vi "Unicode Languages to HEX-String Array.vi"(11 "Config Data in":T1) -> (3 "Config Data out":T1)   [LabVIEW 2019, in "Language Selection.lvlib"]
doc: "- - -\nCopyright (c) 2026, Merecs Engineering GmbH"
uses:
  Language Selection.lvlib
  TypeDefs/Cluster Language Configuration.ctl
  Cluster Settings Data.ctl
  TypeDefs/Cluster Language.ctl
  TypeDefs/Cluster PropertyTranslation.ctl
  TypeDefs/Enum Property Type.ctl
panel:
  # "Connector Pane"
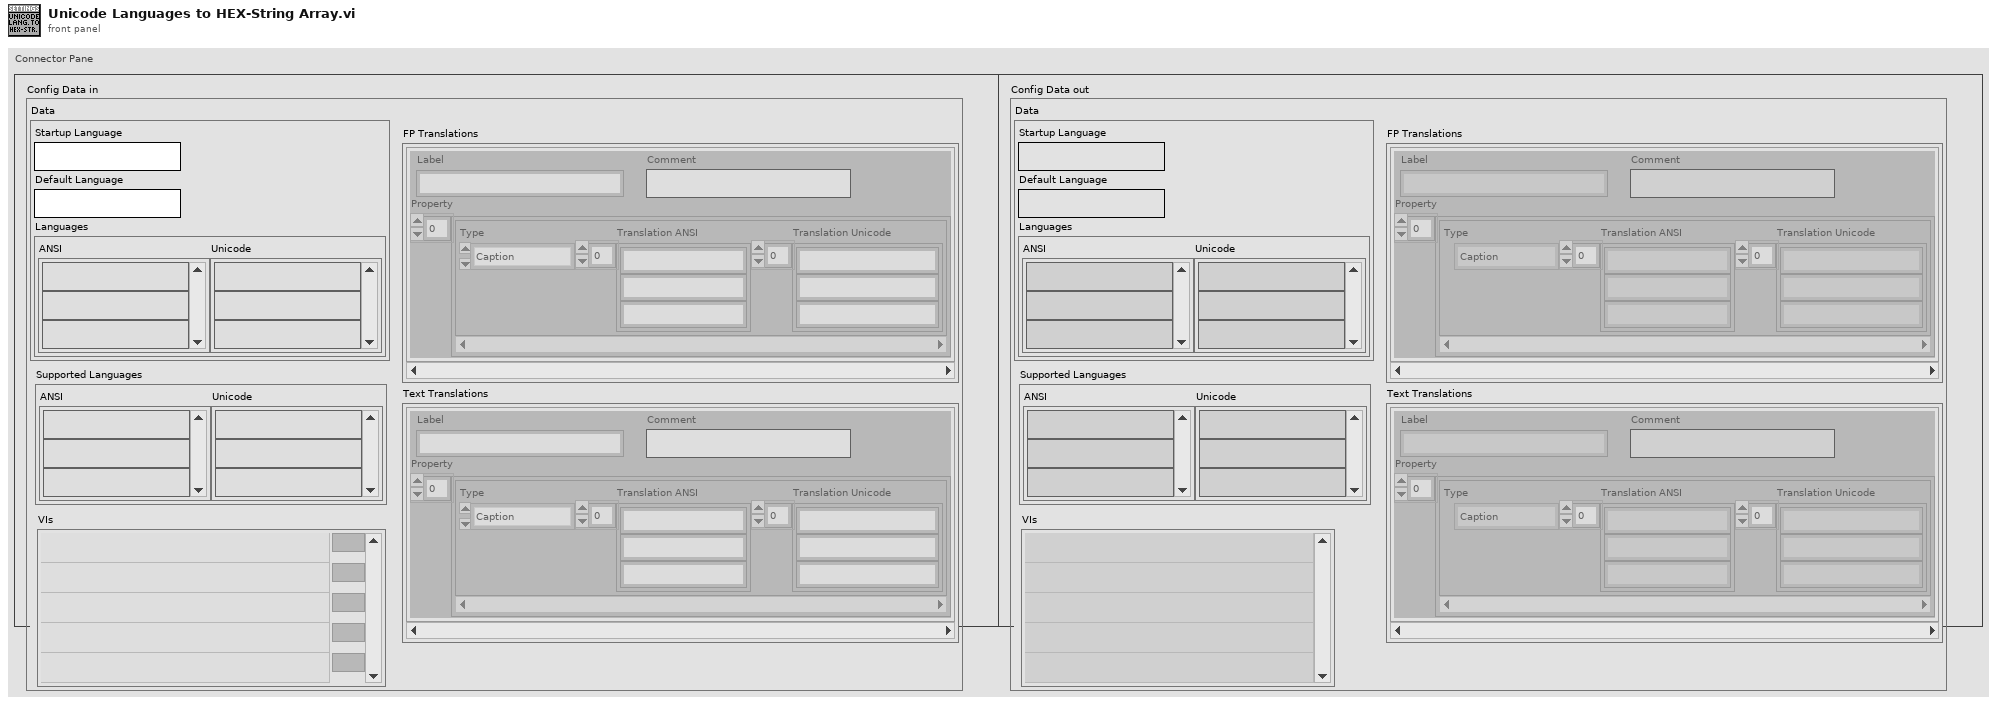
[diagram p1: front panel]
types:
  T1 = typedef "Language Selection.lvlib/Cluster Language Configuration.ctl" = cluster{"Data":T2, "Supported Languages":cluster{"ANSI":string[], "Unicode":string[]}, "VIs":path[], "FP Translations":T3[], "Text Translations":T3[]}
  T2 = typedef "Language Selection.lvlib/Cluster Settings Data.ctl" = cluster{"Startup Language":string, "Default Language":string, "Languages":cluster{"ANSI":string[], "Unicode":string[]}}
  T3 = typedef "Language Selection.lvlib/Cluster Language.ctl" = cluster{"Label":string, "Comment":string, "Property":T4[]}
  T4 = typedef "Language Selection.lvlib/Cluster PropertyTranslation.ctl" = cluster{"Type":T5, "Translation ANSI":string[], "Translation Unicode":string[]}
  T5 = typedef "Language Selection.lvlib/Enum Property Type.ctl" = enum16{"NA", "Caption", "String Value", "Boolean Text", "Ring Strings", "1D Array Elements", "2D Array Elements", "(MC)Listbox Header", "(MC)Listbox Items", "Tab Pages Names", "X & Y GraphChart", "Plot Names", "Table Headers", "Table Items", "TipStrip", "Combobox Strings", "Cursor Name", "Tree Col Headers"}
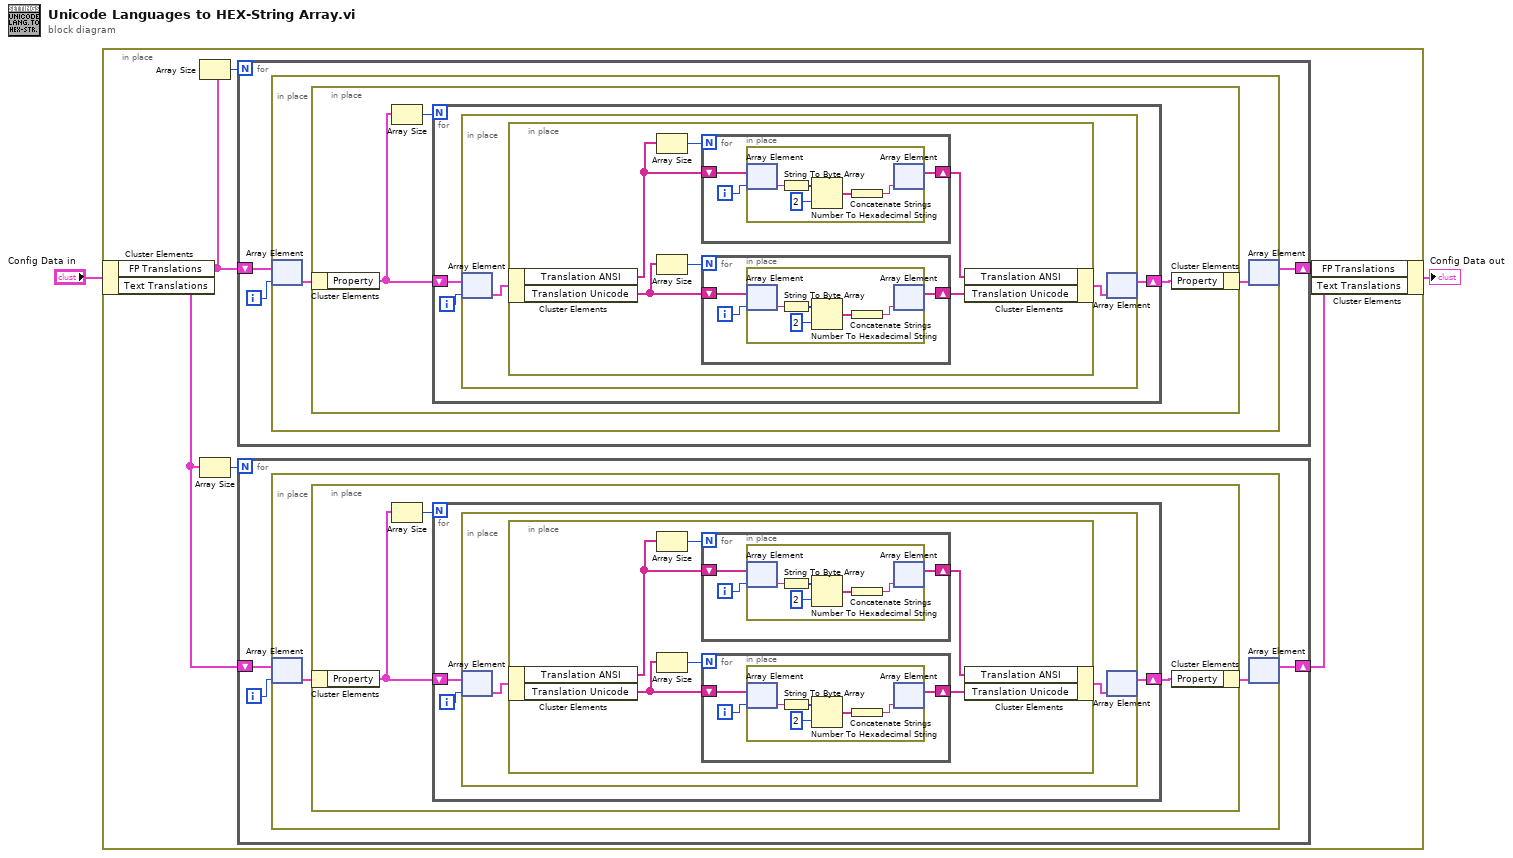
[diagram p0: block diagram]
diagram:
  n1 = in-place {
    n2 = in-place-cluster #1("Config Data in") -> ("FP Translations"=w7:T3[], "Text Translations"=w4:T3[])
    n3 = Array Size(array=w7) -> (size(s)=w8:i32)
    n4 = Array Size(array=w4) -> (size(s)=w5:i32)
    n5 = for {
      N: w8 -> [_]
      shift-right: [w45] -> w6
      shift-left: w7 -> [w46]
      i -> [w44]
      n6 = in-place {
        n7 = in-place-array #2(w46, w44) -> (w48:T3)
        n8 = in-place {
          n9 = in-place-cluster #3(w48) -> ("Property"=w50:T4[])
          n10 = Array Size(array=w50) -> (size(s)=w51:i32)
          n11 = for {
            N: w51 -> [_]
            shift-right: [w52] -> w49
            shift-left: w50 -> [w54]
            i -> [w53]
            n12 = in-place {
              n13 = in-place-array #4(w54, w53) -> (w56:T4)
              n14 = in-place {
                n15 = in-place-cluster #5(w56) -> ("Translation ANSI"=w58:string[], "Translation Unicode"=w62:string[])
                n16 = Array Size(array=w58) -> (size(s)=w59:i32)
                n17 = Array Size(array=w62) -> (size(s)=w61:i32)
                n18 = for {
                  N: w59 -> [_]
                  shift-right: [w63] -> w57
                  shift-left: w58 -> [w65]
                  i -> [w64]
                  n19 = in-place {
                    n20 = in-place-array #6(w65, w64) -> (w68:string)
                    n21 = String To Byte Array(string=w68) -> (unsigned byte array=w70:u8[])
                    n22 = Number To Hexadecimal String(1:i16 2 ("width (-)"), 2:w70) -> (0:w69:string[])
                    n23 = Concatenate Strings(w69) -> (w67:string)
                    n24 = in-place-array #6(w67) -> (w63:string[])  [unwired: 1 out]
                  }
                }
                n25 = for {
                  N: w61 -> [_]
                  shift-right: [w71] -> w60
                  shift-left: w62 -> [w73]
                  i -> [w72]
                  n26 = in-place {
                    n27 = in-place-array #7(w73, w72) -> (w76:string)
                    n28 = String To Byte Array(string=w76) -> (unsigned byte array=w78:u8[])
                    n29 = Number To Hexadecimal String(1:i16 2 ("width (-)"), 2:w78) -> (0:w77:string[])
                    n30 = Concatenate Strings(w77) -> (w75:string)
                    n31 = in-place-array #7(w75) -> (w71:string[])  [unwired: 1 out]
                  }
                }
                n32 = in-place-cluster #5("Translation ANSI"=w57, "Translation Unicode"=w60) -> (w55:T4)
              }
              n33 = in-place-array #4(w55) -> (w52:T4[])  [unwired: 1 out]
            }
          }
          n34 = in-place-cluster #3("Property"=w49) -> (w47:T3)
        }
        n35 = in-place-array #2(w47) -> (w45:T3[])  [unwired: 1 out]
      }
    }
    n36 = for {
      N: w5 -> [_]
      shift-right: [w10] -> w3
      shift-left: w4 -> [w11]
      i -> [w9]
      n37 = in-place {
        n38 = in-place-array #8(w11, w9) -> (w13:T3)
        n39 = in-place {
          n40 = in-place-cluster #9(w13) -> ("Property"=w15:T4[])
          n41 = Array Size(array=w15) -> (size(s)=w16:i32)
          n42 = for {
            N: w16 -> [_]
            shift-right: [w17] -> w14
            shift-left: w15 -> [w19]
            i -> [w18]
            n43 = in-place {
              n44 = in-place-array #10(w19, w18) -> (w21:T4)
              n45 = in-place {
                n46 = in-place-cluster #11(w21) -> ("Translation ANSI"=w23:string[], "Translation Unicode"=w27:string[])
                n47 = Array Size(array=w23) -> (size(s)=w24:i32)
                n48 = Array Size(array=w27) -> (size(s)=w26:i32)
                n49 = for {
                  N: w24 -> [_]
                  shift-right: [w28] -> w22
                  shift-left: w23 -> [w30]
                  i -> [w29]
                  n50 = in-place {
                    n51 = in-place-array #12(w30, w29) -> (w33:string)
                    n52 = String To Byte Array(string=w33) -> (unsigned byte array=w35:u8[])
                    n53 = Number To Hexadecimal String(1:i16 2 ("width (-)"), 2:w35) -> (0:w34:string[])
                    n54 = Concatenate Strings(w34) -> (w32:string)
                    n55 = in-place-array #12(w32) -> (w28:string[])  [unwired: 1 out]
                  }
                }
                n56 = for {
                  N: w26 -> [_]
                  shift-right: [w36] -> w25
                  shift-left: w27 -> [w38]
                  i -> [w37]
                  n57 = in-place {
                    n58 = in-place-array #13(w38, w37) -> (w41:string)
                    n59 = String To Byte Array(string=w41) -> (unsigned byte array=w43:u8[])
                    n60 = Number To Hexadecimal String(1:i16 2 ("width (-)"), 2:w43) -> (0:w42:string[])
                    n61 = Concatenate Strings(w42) -> (w40:string)
                    n62 = in-place-array #13(w40) -> (w36:string[])  [unwired: 1 out]
                  }
                }
                n63 = in-place-cluster #11("Translation ANSI"=w22, "Translation Unicode"=w25) -> (w20:T4)
              }
              n64 = in-place-array #10(w20) -> (w17:T4[])  [unwired: 1 out]
            }
          }
          n65 = in-place-cluster #9("Property"=w14) -> (w12:T3)
        }
        n66 = in-place-array #8(w12) -> (w10:T3[])  [unwired: 1 out]
      }
    }
    n67 = in-place-cluster #1("FP Translations"=w6, "Text Translations"=w3) -> (→"Config Data out":T1)
  }
